vi "Migrate Measurement Dependencies.vi"(0 "Project path":path, 5 "Measurement path":path, 7 "Dependencies path":path[](array[path]), 9 "Plug-in name":string, 11 "error in (no error)":errorcluster) -> (4 "Project reference":refnum<vi>, 6 "MeasurementCore reference":refnum<vi>, 8 "Outside items":string[](array[string]), 15 "error out":errorcluster)   [LabVIEW 2021, in "Multiple Migrator.lvlib"]
uses:
  Multiple Migrator.lvlib
  controls/Library Info.ctl
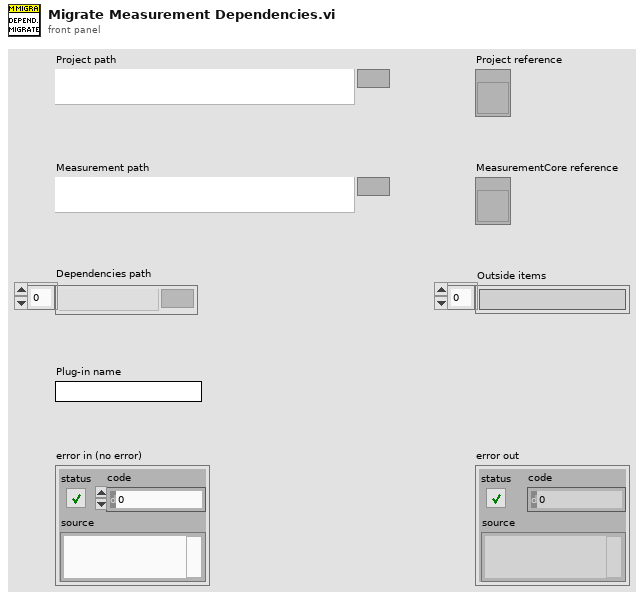
[diagram p1: front panel]
types:
  T1 = typedef "Multiple Migrator.lvlib/Library Info.ctl" = cluster{"Library path":path, "Library name":string}
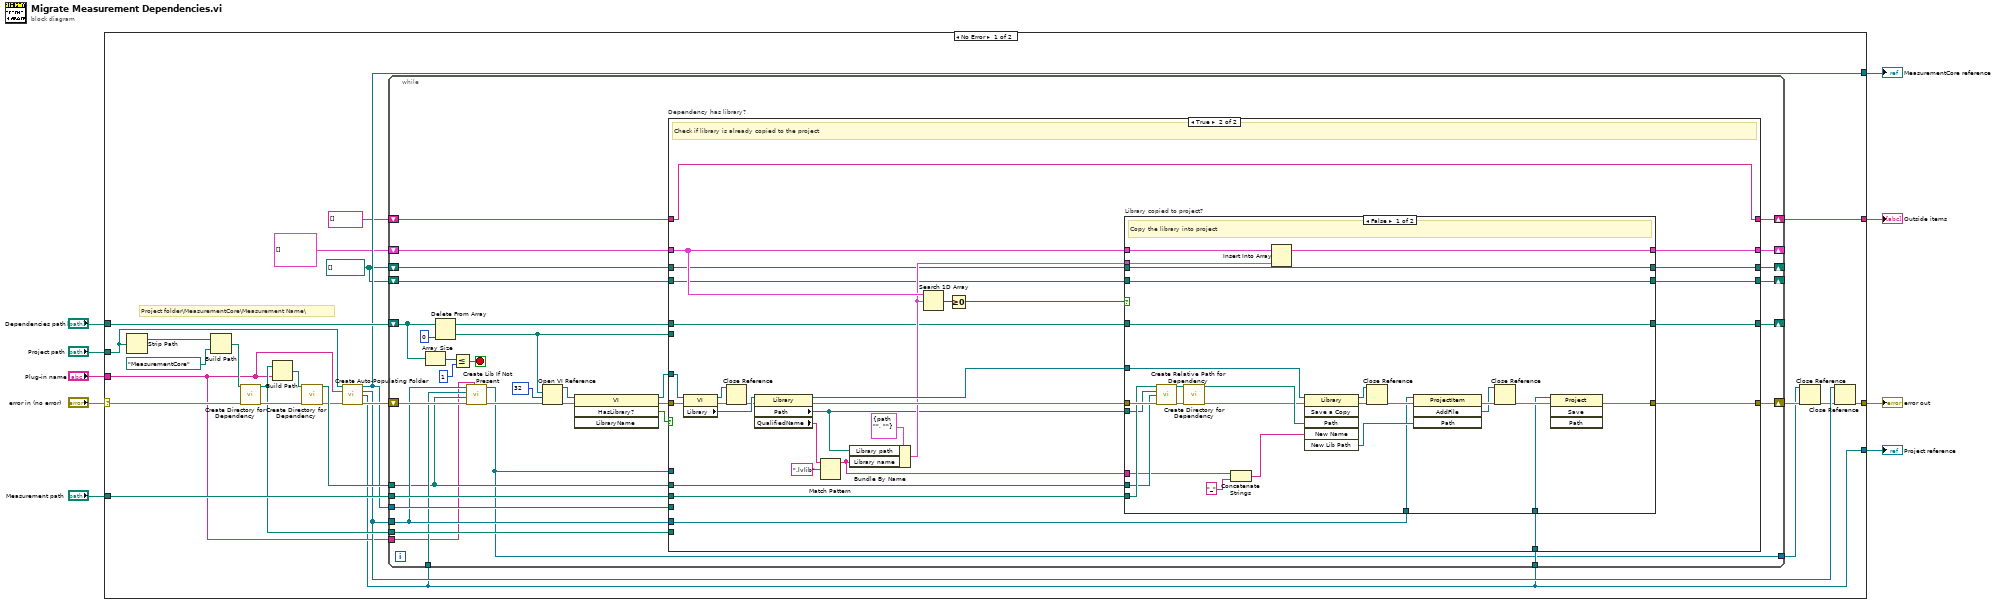
[diagram p0: block diagram]
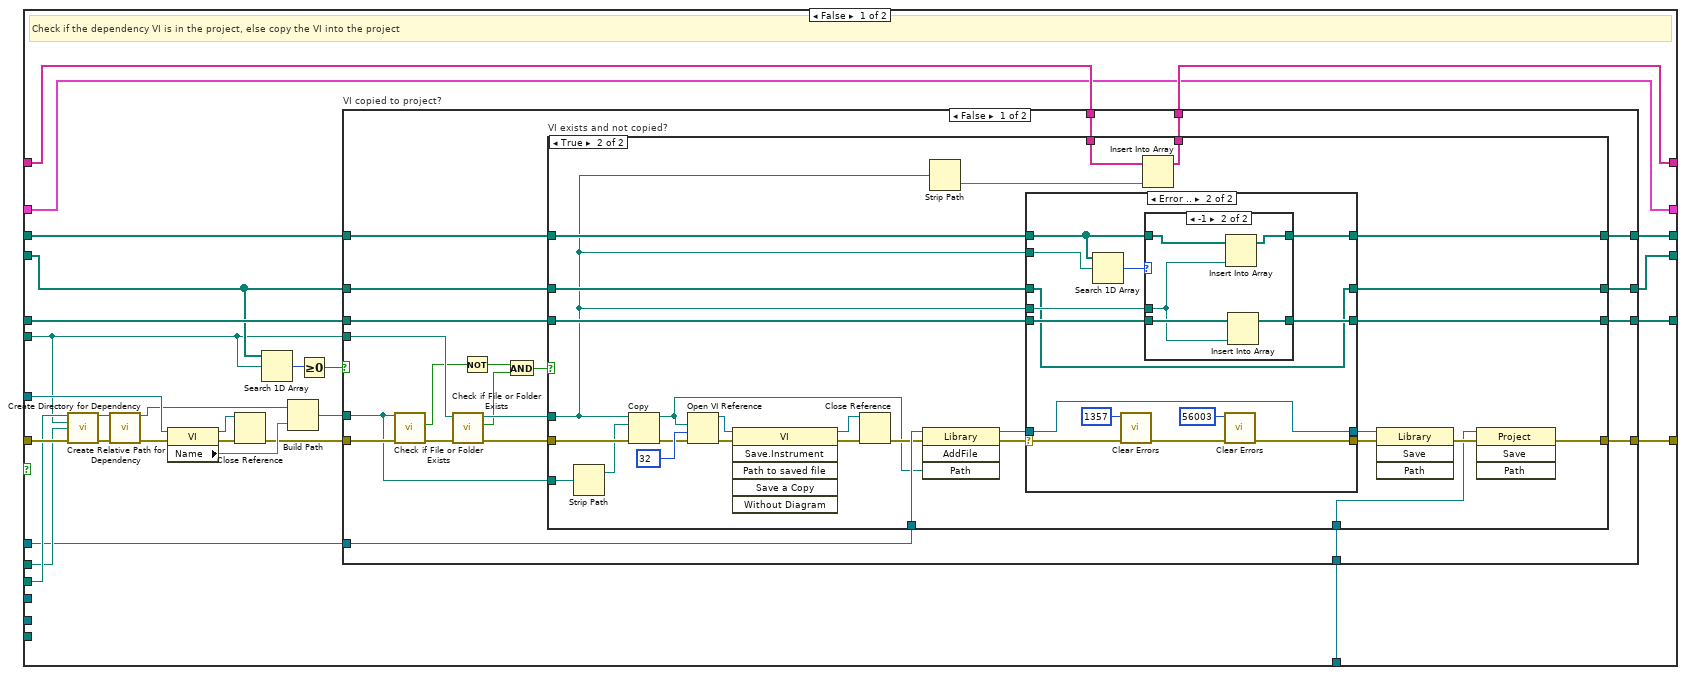
[diagram p2: hidden frame]
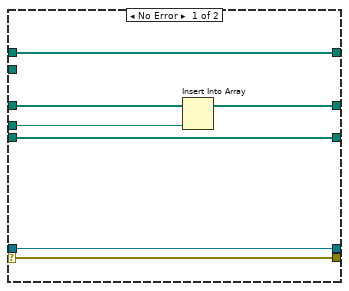
[diagram p4: hidden frame]
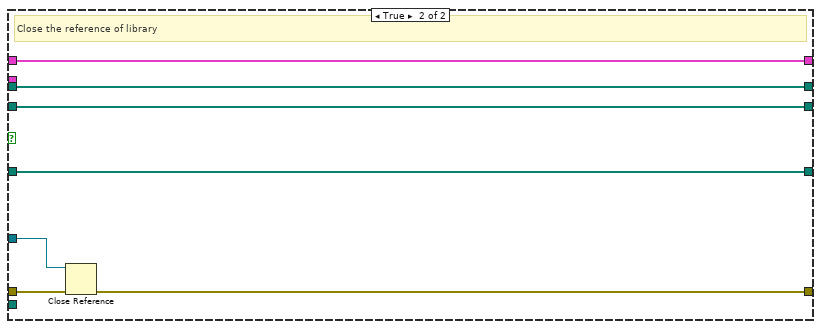
[diagram p7: hidden frame]
diagram:
  n1 = case shown="No Error" "error in (no error)" {
    selector: "error in (no error)" -> [w26 w250]
    tunnel: [w19 w250] -> w8
    tunnel: "Project path" -> [w25 _]
    tunnel: "Measurement path" -> [w30 _]
    tunnel: "Dependencies path" -> [w34 _]
    tunnel: "Plug-in name" -> [w17 _]
    tunnel: [w21 _] -> w3
    tunnel: [w14 _] -> w2
    tunnel: [w15 _] -> w1
    frame No Error {
      w10 = path[] []
      # "Project folder\\MeasurementCore\\Measurement Name\\"
      n2 = Strip Path(path=w25) -> (stripped path=w29:path)  [unwired: 1 out]
      n3 = Build Path(base path=w29, name or relative path=path "MeasurementCore") -> (appended path=w27:path)
      n4 = call "Create Directory for Dependency.vi"("Directory path"=w27, "error in (no error)"=w26) -> ("Directory path out"=w20:path, "error out"=w24:errorcluster)  [unwired: 12 in]
      n5 = Build Path(base path=w20, name or relative path=w17) -> (appended path=w33:path)
      n6 = call "Create Directory for Dependency.vi"("Directory path"=w33, "error in (no error)"=w24) -> ("Directory path out"=w32:path, "error out"=w23:errorcluster)  [unwired: 12 in]
      n7 = call "Create Auto-Populating Folder.vi"("Project path"=w25, "Plug-in name"=w17, "error in (no error)"=w23) -> ("MeasurementCore reference"=w21:refnum<vi>, "Folder reference"=w18:refnum<vi>, "Project reference"=w14:refnum<vi>, "error out"=w22:errorcluster)  [unwired: 9 in]
      n8 = while {
        shift-right: [w56] -> w31
        shift-left: w22 -> [w44]
        shift-right: [w49] -> _
        shift-left: w34 -> [w66]
        tunnel: w32 -> [w40]
        shift-right: [w55] -> _
        shift-left: T1[] [] -> [w58]
        tunnel: w30 -> [w54]
        shift-right: [w51] -> _
        shift-left: w10 -> [w52]
        tunnel: w21 -> [w48]
        tunnel: w20 -> [w47]
        tunnel: w18 -> [w42]
        tunnel: w17 -> [w39]
        shift-right: [w45] -> w15
        shift-left: string[] [] -> [w46]
        tunnel: w14 -> [w41]
        tunnel: w14 -> [w38]
        shift-right: [w37] -> _
        shift-left: w10 -> [w36]
        tunnel: [w35] -> w12
        stop <- w65 stop-if-true
        n9 = Array Size(array=w66) -> (size(s)=w68:i32)
        n10 = Delete From Array(array=w66, index=0) -> (deleted portion=w53:path, array with subset deleted=w50:path[])  [unwired: 1 in]
        n11 = Less Or Equal?(x=w68, y=1) -> (x <= y?=w65:bool)
        n12 = call "Create Lib If Not Present.vi"("Plug-in name"=w39, "error in (no error)"=w44, "DestDirectory"=w40, "ProjectRef"=w41, "VirtualFolderRef"=w42) -> ("error out"=w43:errorcluster, "Library Refnum"=w35:refnum<vi>)  [unwired: 5 in]
        n13 = Open VI Reference(vi path=w53, options=32, error in (no error)=w43) -> (vi reference=w62:refnum<vi>, error out=w64:errorcluster)  [unwired: 3 in]
        n14 = invoke class="VI" method="HasLibrary?"(reference=w62, error in=w64) -> (reference out=w59:refnum<vi>, error out=w60:errorcluster, "Has Library?"=w61:bool)  [unwired: 2 in, 1 out]
        n15 = case "Dependency has library?" shown="True" w61 {
          tunnel: w60 -> [w95 w213]
          tunnel: w59 -> [w91 w214]
          tunnel: w58 -> [w72 w201]
          tunnel: [w86 w202] -> w56
          tunnel: [w72 w200] -> w55
          tunnel: w54 -> [w94 w198]
          tunnel: w40 -> [w77 w196]
          tunnel: w53 -> [w81 _]
          tunnel: w52 -> [w82 w193]
          tunnel: [w76 w192] -> w51
          tunnel: w50 -> [w85 w191]
          tunnel: [w84 w190] -> w49
          tunnel: w48 -> [_ _]
          tunnel: w47 -> [_ _]
          tunnel: w42 -> [_ w189]
          tunnel: w46 -> [w74 w188]
          tunnel: [w73 w188] -> w45
          tunnel: w35 -> [w75 _]
          tunnel: w38 -> [w69 w187]
          tunnel: [w71 w185] -> w37
          tunnel: w36 -> [w70 w186]
          frame False {
            # "Check if the dependency VI is in the project, else copy the VI into the project"
            n16 = call "Create Relative Path for Dependency.vi"("Old Main Path"=w94, "Old Dependency Path"=w81, "New Dir"=w77, "error in (no error)"=w95) -> ("Directory"=w93:path, "error out"=w96:errorcluster)  [unwired: 10 in]
            n17 = call "Create Directory for Dependency.vi"("Directory path"=w93, "error in (no error)"=w96) -> ("Directory path out"=w83:path, "error out"=w92:errorcluster)  [unwired: 12 in]
            n18 = property class="VI"(reference=w91, error in=w92) -> (reference out=w87:refnum<vi>, error out=w90:errorcluster, "Name"=w89:string)
            n19 = Close Reference(reference=w87, error in (no error)=w90) -> (error out=w88:errorcluster)
            n20 = Search 1D Array(1D array=w82, element=w81) -> (index of element=w80:i32)  [unwired: 1 in]
            n21 = Build Path(base path=w83, name or relative path=w89) -> (appended path=w79:path)
            n22 = Greater Or Equal To 0?(x=w80) -> (x >= 0?=w78:bool)
            n23 = case "VI copied to project?" shown="False" w78 {
              tunnel: w88 -> [w117 w184]
              tunnel: w81 -> [w116 _]
              tunnel: [w113 w184] -> w86
              tunnel: w82 -> [w112 w183]
              tunnel: [w111 w183] -> w76
              tunnel: w79 -> [w107 _]
              tunnel: w85 -> [w110 w182]
              tunnel: [w109 w182] -> w84
              tunnel: w74 -> [w102 w181]
              tunnel: [w101 w181] -> w73
              tunnel: w75 -> [w100 _]
              tunnel: [w99 w180] -> w71
              tunnel: w70 -> [w98 w180]
              tunnel: w69 -> [w97 _]
              frame False {
                n24 = call <vilib>:"Check if File or Folder Exists.vi"("error in (no error)"=w117, "path"=w107) -> ("error out"=w108:errorcluster, "file or folder exists?"=w106:bool)  [unwired: 7 in, 1 out]
                n25 = call <vilib>:"Check if File or Folder Exists.vi"("error in (no error)"=w108, "path"=w116) -> ("error out"=w115:errorcluster, "file or folder exists?"=w104:bool, "dup path"=w114:path)  [unwired: 7 in]
                n26 = Not(x=w106) -> (.not. x?=w105:bool)
                n27 = And(x=w105, y=w104) -> (x .and. y?=w103:bool)
                n28 = case "VI exists and not copied?" shown="True" w103 {
                  tunnel: w115 -> [w122 w151]
                  tunnel: w114 -> [_ w131]
                  tunnel: [w122 w133] -> w113
                  tunnel: w112 -> [w121 w150]
                  tunnel: [w121 w149] -> w111
                  tunnel: w107 -> [_ w146]
                  tunnel: w110 -> [w120 w135]
                  tunnel: [w120 w134] -> w109
                  tunnel: w102 -> [w119 w145]
                  tunnel: [w119 w143] -> w101
                  tunnel: w100 -> [_ w142]
                  tunnel: [w118 w141] -> w99
                  tunnel: w98 -> [w118 w140]
                  tunnel: w97 -> [_ w132]
                  frame False {
                  }
                  frame True {
                    n29 = Strip Path(path=w146) -> (stripped path=w148:path)  [unwired: 1 out]
                    n30 = Copy(8:w151, 10:w148, 11:w131) -> (0:w125:errorcluster, 3:w123:path)  [unwired: 2 in, 1 out]
                    n31 = Open VI Reference(vi path=w123, options=32, error in (no error)=w125) -> (vi reference=w128:refnum<vi>, error out=w129:errorcluster)  [unwired: 3 in]
                    n32 = invoke class="VI" method="Save.Instrument"(reference=w128, error in=w129) -> (reference out=w126:refnum<vi>, error out=w127:errorcluster)  [unwired: 4 in, 4 out]
                    n33 = Close Reference(reference=w126, error in (no error)=w127) -> (error out=w124:errorcluster)
                    n34 = invoke class="Library" method="AddFile"(reference=w142, error in=w124, "Path"=w123) -> (reference out=w139:refnum<vi>, error out=w138:errorcluster)  [unwired: 1 in, 2 out]
                    n35 = Strip Path(path=w131) -> (name=w144:string)  [unwired: 1 out]
                    n36 = case shown="Error .." w138 {
                      selector: w138 -> [w153 w172]
                      tunnel: w150 -> [w158 w159]
                      tunnel: [w157 w159] -> w149
                      tunnel: w131 -> [w156 w162]
                      tunnel: [w155 w163] -> w141
                      tunnel: w140 -> [w155 w164]
                      tunnel: [w154 w161] -> w136
                      tunnel: w139 -> [w154 w161]
                      tunnel: [w153 w170] -> w137
                      tunnel: w135 -> [w152 w166]
                      tunnel: [w152 w165] -> w134
                      tunnel: w131 -> [_ w167]
                      frame No Error {
                        n37 = Insert Into Array(array=w158, new element=w156) -> (w157:path[])  [unwired: 1 in]
                      }
                      frame Error {
                        n38 = Search 1D Array(1D array=w164, element=w167) -> (index of element=w160:i32)  [unwired: 1 in]
                        n39 = call <vilib>:"Clear Errors.vi"("error in (no error)"=w172, "specific error code to clear (0: all)"=1357) -> ("error out"=w171:errorcluster)  [unwired: 4 in, 1 out]
                        n40 = case shown="-1" w160 {
                          tunnel: w166 -> [w173 w179]
                          tunnel: [w173 w178] -> w165
                          tunnel: w164 -> [w174 w177]
                          tunnel: [w174 w176] -> w163
                          tunnel: w162 -> [_ w175]
                          frame Default {
                          }
                          frame -1 {
                            n41 = Insert Into Array(array=w177, new element=w175) -> (w176:path[])  [unwired: 1 in]
                            n42 = Insert Into Array(array=w179, new element=w175) -> (w178:path[])  [unwired: 1 in]
                          }
                        }
                        n43 = call <vilib>:"Clear Errors.vi"("error in (no error)"=w171, "specific error code to clear (0: all)"=56003) -> ("error out"=w170:errorcluster)  [unwired: 4 in, 1 out]
                      }
                    }
                    n44 = Insert Into Array(array=w145, new element=w144) -> (w143:string[])  [unwired: 1 in]
                    n45 = invoke class="Library" method="Save"(reference=w136, error in=w137) -> (error out=w147:errorcluster)  [unwired: 2 in, 3 out]
                    n46 = invoke class="Project" method="Save"(reference=w132, error in=w147) -> (error out=w133:errorcluster)  [unwired: 2 in, 3 out]
                  }
                }
              }
              frame True {
              }
            }
          }
          frame True {
            # "Check if library is already copied to the project"
            n47 = property class="VI"(reference=w214, error in=w213) -> (reference out=w204:refnum<vi>, error out=w212:errorcluster, "Library"=w211:refnum<vi>)
            n48 = Close Reference(reference=w204, error in (no error)=w212) -> (error out=w205:errorcluster)
            n49 = property class="Library"(reference=w211, error in=w205) -> (reference out=w203:refnum<vi>, error out=w206:errorcluster, "Path"=w197:path, "QualifiedName"=w207:string)
            n50 = Match Pattern(string=w207, regular expression=".lvlib") -> (before substring=w194:string)  [unwired: 1 in, 3 out]
            n51 = Bundle By Name(cluster=T1 {"Library path"=path "", "Library name"=""} ("Cluster"), "Library path"=w197, "Library name"=w194) -> (w199:T1)
            n52 = Search 1D Array(1D array=w201, element=w199) -> (index of element=w209:i32)  [unwired: 1 in]
            n53 = Greater Or Equal To 0?(x=w209) -> (x >= 0?=w208:bool)
            n54 = case "Library copied to project?" shown="False" w208 {
              tunnel: w206 -> [w237 w248]
              tunnel: w203 -> [w230 w249]
              tunnel: [w217 w247] -> w202
              tunnel: w201 -> [w242 w246]
              tunnel: [w241 w246] -> w200
              tunnel: w199 -> [w240 _]
              tunnel: w198 -> [w236 _]
              tunnel: w197 -> [w235 _]
              tunnel: w196 -> [w234 _]
              tunnel: w194 -> [w220 _]
              tunnel: w193 -> [w227 w245]
              tunnel: [w227 w245] -> w192
              tunnel: [w226 w244] -> w190
              tunnel: w191 -> [w226 w244]
              tunnel: w189 -> [w221 _]
              tunnel: w187 -> [w216 _]
              tunnel: [w215 w243] -> w185
              tunnel: w186 -> [w215 w243]
              frame False {
                # "Copy the library into project"
                n55 = call "Create Relative Path for Dependency.vi"("Old Main Path"=w236, "Old Dependency Path"=w235, "New Dir"=w234, "error in (no error)"=w237) -> ("Directory"=w232:path, "error out"=w233:errorcluster)  [unwired: 10 in]
                n56 = call "Create Directory for Dependency.vi"("Directory path"=w232, "error in (no error)"=w233) -> ("Directory path out"=w231:path, "error out"=w229:errorcluster)  [unwired: 12 in]
                n57 = Concatenate Strings(w220, "_" ("string")) -> (w218:string)
                n58 = Insert Into Array(array=w242, new element=w240) -> (w241:T1[])  [unwired: 1 in]
                n59 = invoke class="Library" method="Save a Copy"(reference=w230, error in=w229, "Path"=w231, "New Name"=w218) -> (reference out=w238:refnum<vi>, error out=w239:errorcluster, "New Lib Path"=w224:path)  [unwired: 2 in, 3 out]
                n60 = Close Reference(reference=w238, error in (no error)=w239) -> (error out=w228:errorcluster)
                n61 = invoke class="ProjectItem" method="AddFile"(reference=w221, error in=w228, "Path"=w224) -> (error out=w225:errorcluster, "AddFile"=w222:refnum<vi>)  [unwired: 1 in, 2 out]
                n62 = Close Reference(reference=w222, error in (no error)=w225) -> (error out=w223:errorcluster)
                n63 = invoke class="Project" method="Save"(reference=w216, error in=w223) -> (error out=w217:errorcluster)  [unwired: 2 in, 3 out]
              }
              frame True {
                # "Close the reference of library"
                n64 = Close Reference(reference=w249, error in (no error)=w248) -> (error out=w247:errorcluster)
              }
            }
          }
        }
      }
      n65 = Close Reference(reference=w12, error in (no error)=w31) -> (error out=w13:errorcluster)
      n66 = Close Reference(reference=w18, error in (no error)=w13) -> (error out=w19:errorcluster)
    }
    frame Error {
    }
  }
  "error out" <- w8
  "MeasurementCore reference" <- w3
  "Project reference" <- w2
  "Outside items" <- w1
